vi "Command Type.vi"(11 "Stop Seq Command Config in":refnum<class "Stop Seq Command Config.lvclass">) -> (2 "Command Type":T1)   [LabVIEW 2020, in "VolatusSeqConfig.lvlib" / "Stop Seq Command Config.lvclass"]
uses:
  Stop Seq Command Config.lvclass
  Stop Seq Command Config.lvclass/Stop Seq Command Config.ctl
  Command Type.ctl
  VolatusSeqConfig.lvlib
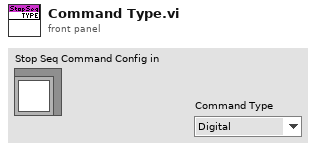
[diagram p1: front panel]
types:
  T1 = typedef "VolatusSeqConfig.lvlib/Command Type.ctl" = enum16{"Digital", "Numeric", "Transition", "Stop", "StartLog", "StopLog"}
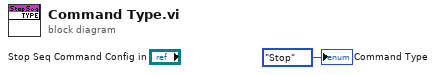
[diagram p0: block diagram]
diagram:
  "Command Type" <- Command_Type."Stop" ("Command Type")
